vi "Delete User.vi"(5 "Save File":bool=TRUE, 6 "error in (no error)":errorcluster, 8 "LoginName":string, 9 "EasyUserManager in":refnum<class "EasyUserManager.lvclass">) -> (0 "error out":errorcluster, 3 "EasyUserManager out":refnum<class "EasyUserManager.lvclass">)   [LabVIEW 2024, in "EasyUserManager.lvclass"]
doc: "Delete the user specified by <B>LoginName</B>. The user is also removed from all groups. \n\n<B>Note:</B> This VI will display a warning and abort if there is only one user available. \n\nThe boolean input <B>Save File</B> controls whether changes are immediately saved to the users file (Default: True)."
uses:
  EasyUserManager.lvclass
  EasyUserManager.lvclass/EasyUserManager.ctl
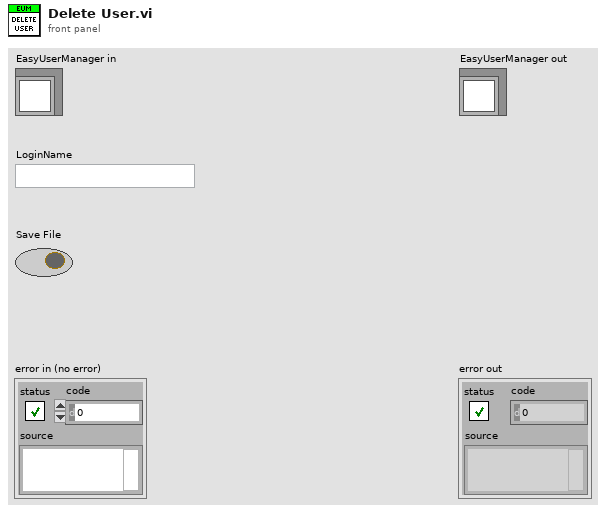
[diagram p1: front panel]
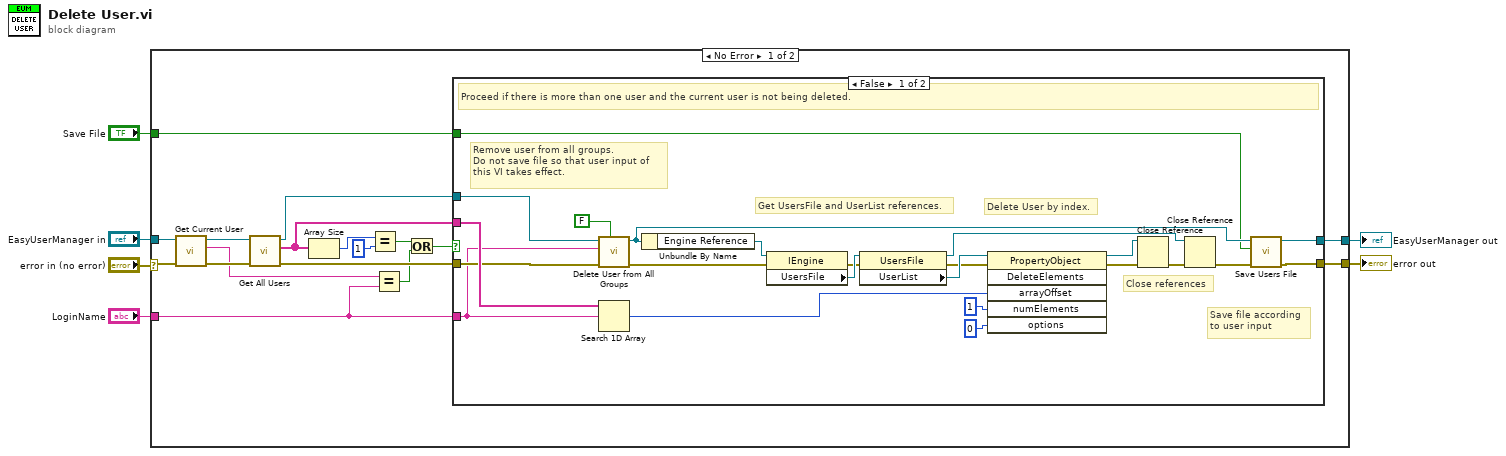
[diagram p0: block diagram]
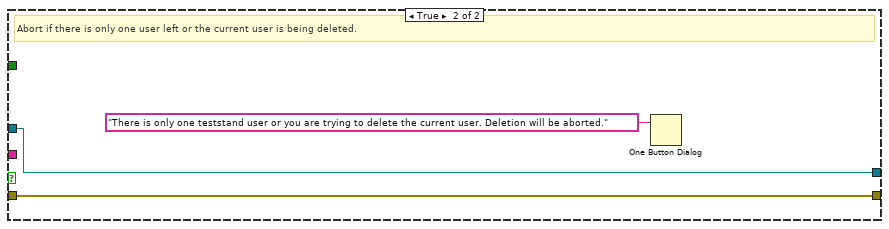
[diagram p2: hidden frame]
diagram:
  n1 = case shown="No Error" "error in (no error)" {
    selector: "error in (no error)" -> [w14 w51]
    tunnel: [w18 w51] -> w5
    tunnel: [w19 w50] -> w3
    tunnel: "EasyUserManager in" -> [w15 w50]
    tunnel: "Save File" -> [w8 _]
    tunnel: "LoginName" -> [w7 _]
    frame No Error {
      n2 = call "Get Current User.vi"("error in (no error)"=w14, "EasyUserManager in"=w15) -> ("error out"=w13:errorcluster, "LoginName"=w11:string, "EasyUserManager out"=w16:refnum<class "EasyUserManager.lvclass">)  [unwired: 3 in]
      n3 = call "Get All Users.vi"("error in (no error)"=w13, "EasyUserManager in"=w16) -> ("error out"=w17:errorcluster, "Users"=w23:string[], "EasyUserManager out"=w20:refnum<class "EasyUserManager.lvclass">)  [unwired: 3 in]
      n4 = Array Size(array=w23) -> (size(s)=w22:i32)
      n5 = Equal?(x=w22, y=1) -> (x = y?=w12:bool)
      n6 = Equal?(x=w11, y=w7) -> (x = y?=w10:bool)
      n7 = Or(x=w12, y=w10) -> (x .or. y?=w9:bool)
      n8 = case shown="False" w9 {
        tunnel: w23 -> [w46 _]
        tunnel: w20 -> [w30 w48]
        tunnel: [w33 w48] -> w19
        tunnel: [w31 w47] -> w18
        tunnel: w17 -> [w28 w47]
        tunnel: w7 -> [w26 _]
        tunnel: w8 -> [w24 _]
        frame False {
          # "Delete User by index."
          # "Get UsersFile and UserList references."
          # "Remove user from all groups.\nDo not save file so that user input of \nthis VI takes effect."
          # "Save file according\nto user input"
          # "Close references"
          # "Proceed if there is more than one user and the current user is not being deleted."
          n9 = call "Delete User from All Groups.vi"("Save File"=FALSE, "error in (no error)"=w28, "LoginName"=w26, "EasyUserManager in"=w30) -> ("error out"=w27:errorcluster, "EasyUserManager out"=w29:refnum<class "EasyUserManager.lvclass">)  [unwired: 4 in]
          n10 = Search 1D Array(1D array=w46, element=w26) -> (index of element=w39:i32)  [unwired: 1 in]
          n11 = Unbundle By Name(w29) -> ("Engine Reference"=w43:refnum<k7>)
          n12 = property on="Property Node" class="IEngine"(reference=w43, error in=w27) -> (error out=w44:errorcluster, "UsersFile"=w45:refnum<k7>)  [unwired: 1 out]
          n13 = property on="Property Node" class="UsersFile"(reference=w45, error in=w44) -> (reference out=w36:refnum<k7>, error out=w38:errorcluster, "UserList"=w40:refnum<k7>)
          n14 = invoke on="Invoke Node" class="PropertyObject" method="DeleteElements"(reference=w40, error in=w38, "arrayOffset"=w39, "numElements"=1, "options"=0) -> (reference out=w37:refnum<k7>, error out=w34:errorcluster)  [unwired: 1 in, 4 out]
          n15 = Close Reference(reference=w37, error in (no error)=w34) -> (error out=w35:errorcluster)
          n16 = Close Reference(reference=w36, error in (no error)=w35) -> (error out=w32:errorcluster)
          n17 = call "Save Users File.vi"("error in (no error)"=w32, "Save"=w24, "EasyUserManager in"=w29) -> ("error out"=w31:errorcluster, "EasyUserManager out"=w33:refnum<class "EasyUserManager.lvclass">)  [unwired: 3 in]
        }
        frame True {
          # "Abort if there is only one user left or the current user is being deleted."
          n18 = One Button Dialog(message="There is only one teststand user or you are trying to delete the current user. Deletion will be aborted.") -> ()  [unwired: 1 in, 1 out]
        }
      }
    }
    frame Error {
      # "Pass error and do nothing."
    }
  }
  "error out" <- w5
  "EasyUserManager out" <- w3
